vi "Abbreviations.vi"() -> ()   [LabVIEW 2020, in "Silly Billy.lvlib"]
uses:
  Silly Billy.lvlib
panel:
  in  "Abbreviations":cluster{"word":string, "abbreviation":string}[](array[cluster])=[{"word"="_", "abbreviation"=" "}, {"word"="labview", "abbreviation"="lv"}, {"word"="message", "abbreviation"="msg"}]
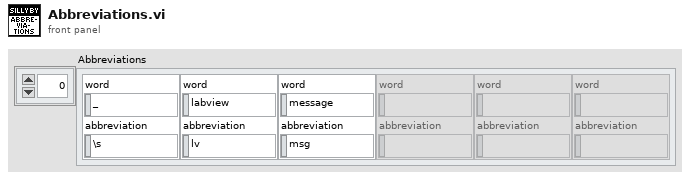
[diagram p1: front panel]
diagram:
